vi "connectToServer.vi"(8 "error in (no error)":errorcluster, 11 "server":string) -> (0 "error out":errorcluster)   [LabVIEW 2018, in "ThirdPartyYoutubeClass.lvclass"]
uses:
  ThirdPartyYoutubeClass.lvclass
  ConsoleOut/Print Options.ctl
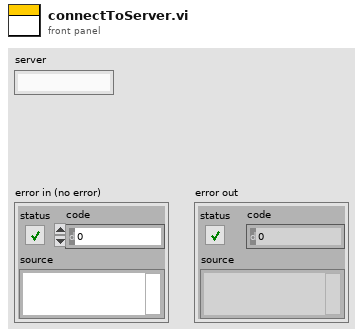
[diagram p1: front panel]
types:
  T1 = typedef "Print Options.ctl" = enum16{"Create", "Get Reference", "Print", "Print Header", "Close"}
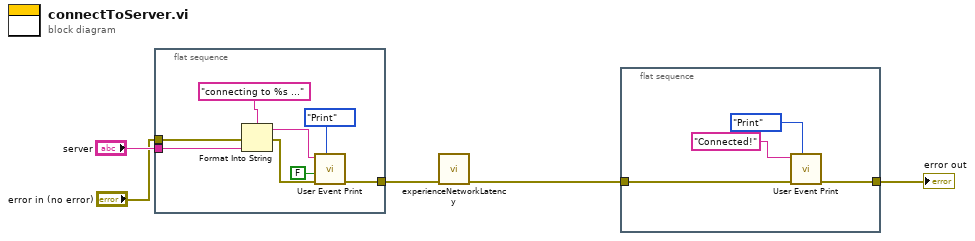
[diagram p0: block diagram]
diagram:
  n1 = flat-sequence {
    tunnel: "server" -> [w12]
    tunnel: [w9] -> w4
    tunnel: "error in (no error)" -> [w10]
    frame #0 {
      n2 = Format Into String(format string="connecting to %s ..." ("ConsoleOut"), error in=w10, w12) -> (resulting string=w8:string, error out=w11:errorcluster)  [unwired: 1 in]
      n3 = call "User Event Print.vi"("Options"=Print_Options."Print", "error in (no error)"=w11, "add EOL? (T)"=FALSE, "String to Print"=w8) -> ("error out"=w9:errorcluster)  [unwired: 6 in, 1 out]
    }
  }
  n4 = call "experienceNetworkLatency.vi"("error in (no error)"=w4) -> ("error out"=w3:errorcluster)  [unwired: 10 in]
  n5 = flat-sequence {
    tunnel: w3 -> [w17]
    tunnel: [w16] -> w1
    frame #0 {
      n6 = call "User Event Print.vi"("Options"=Print_Options."Print", "error in (no error)"=w17, "String to Print"="Connected!" ("ConsoleOut")) -> ("error out"=w16:errorcluster)  [unwired: 7 in, 1 out]
    }
  }
  "error out" <- w1
